vi "Stock Names.vi"() -> (3 "names":string[](array[string]))   [LabVIEW 2020, in "Full Featured MCP Server.lvlib"]
doc: "Returns the names of all stocks, in the order of the Stock Catalogue."
uses:
  Full Featured MCP Server.lvlib
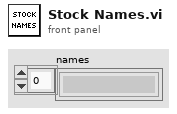
[diagram p1: front panel]
types:
  T1 = cluster{"name":string, "sector":i32, "quality":i32, "start price":dbl, "drift":dbl, "volatility":dbl, "beta":dbl, "jumpiness":dbl, "description":string}[]
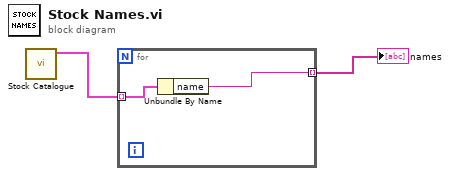
[diagram p0: block diagram]
diagram:
  n1 = call "Stock Catalogue.vi"() -> ("stocks"=w1:T1)  [unwired: 10 in, 1 out]
  n2 = for {
    tunnel: w1 -> [w3] mode=indexing
    tunnel: [w4] -> w2 mode=indexing
    n3 = Unbundle By Name(w3) -> ("name"=w4:string)
  }
  "names" <- w2
